vi "Wire Handle Messages Case.vi"(8 "error in (no error)":errorcluster, 11 "Getter Generator in":refnum<class "Getter Generator.lvclass">) -> (0 "error out":errorcluster, 3 "Getter Generator out":refnum<class "Getter Generator.lvclass">)   [LabVIEW 2020, in "Method Generation.lvlib" / "Getter Generator.lvclass"]
uses:
  Getter Generator.lvclass
  Getter Generator.lvclass/Getter Generator.ctl
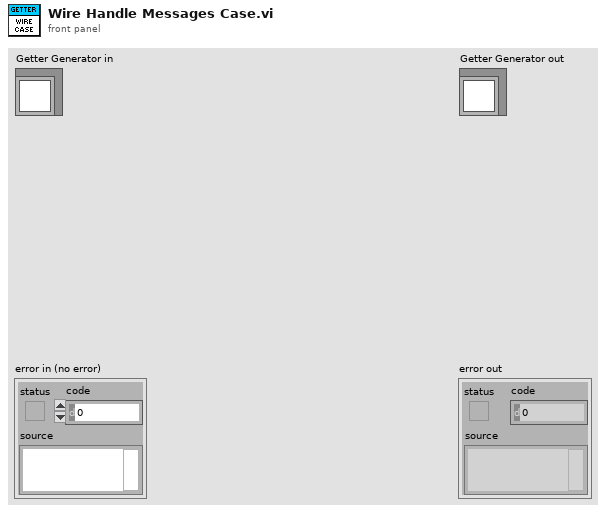
[diagram p1: front panel]
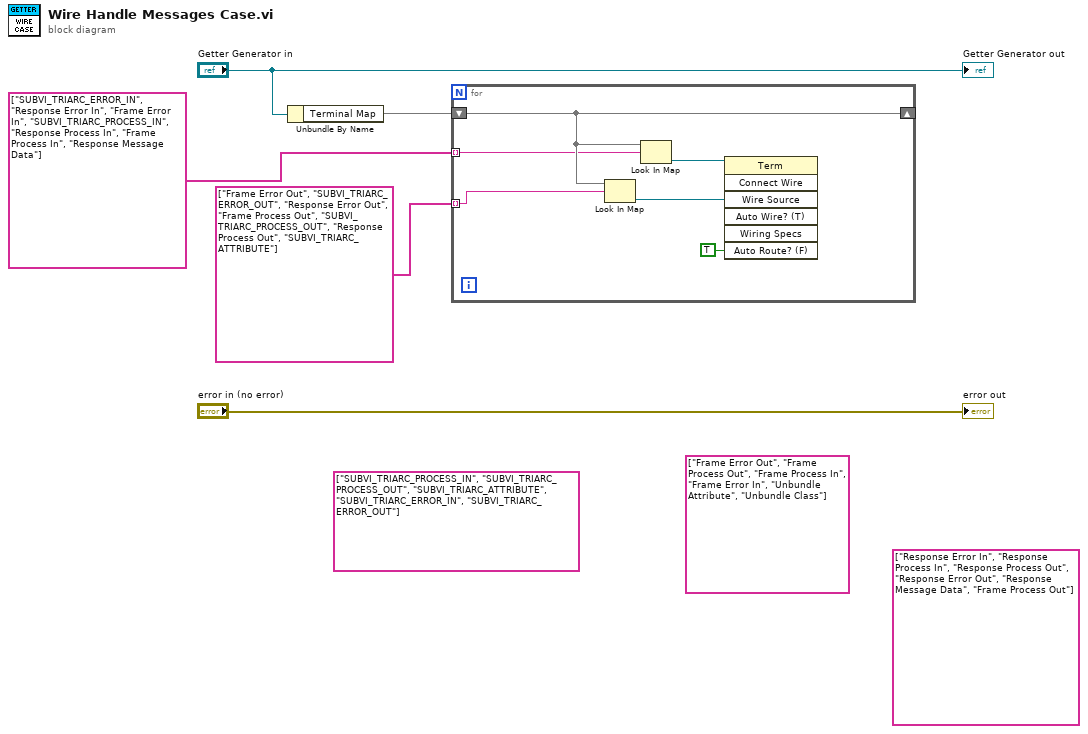
[diagram p0: block diagram]
diagram:
  (unwired) string[] ["Response Error In", "Response Process In", "Response Process Out", "Response Error Out", "Response Message Data", "Frame Process Out"] ("key")
  (unwired) string[] ["Frame Error Out", "Frame Process Out", "Frame Process In", "Frame Error In", "Unbundle Attribute", "Unbundle Class"] ("key")
  (unwired) string[] ["SUBVI_TRIARC_PROCESS_IN", "SUBVI_TRIARC_PROCESS_OUT", "SUBVI_TRIARC_ATTRIBUTE", "SUBVI_TRIARC_ERROR_IN", "SUBVI_TRIARC_ERROR_OUT"]
  n1 = Unbundle By Name("Getter Generator in") -> ("Terminal Map"=w3:map{string, refnum<vi>})
  n2 = for {
    shift-right: [w11] -> _
    shift-left: w3 -> [w11]
    tunnel: string[] ["SUBVI_TRIARC_ERROR_IN", "Response Error In", "Frame Error In", "SUBVI_TRIARC_PROCESS_IN", "Response Process In", "Frame Process In", "Response Message Data"] ("key") -> [w10] mode=indexing
    tunnel: string[] ["Frame Error Out", "SUBVI_TRIARC_ERROR_OUT", "Response Error Out", "Frame Process Out", "SUBVI_TRIARC_PROCESS_OUT", "Response Process Out", "SUBVI_TRIARC_ATTRIBUTE"] ("key") -> [w9] mode=indexing
    n3 = Look In Map(map=w11, key=w9) -> (value=w7:refnum<vi>)  [unwired: 1 in, 1 out]
    n4 = Look In Map(map=w11, key=w10) -> (value=w8:refnum<vi>)  [unwired: 1 in, 1 out]
    n5 = invoke class="Term" method="Connect Wire"(reference=w8, "Wire Source"=w7, "Auto Route? (F)"=TRUE) -> ()  [unwired: 4 in, 7 out]
  }
  "error out" <- "error in (no error)"
  "Getter Generator out" <- "Getter Generator in"
